vi "fix_shared_library_wildcards.vi"(8 "error in (no error)":errorcluster, 11 "UnpackedPackage in":refnum<class "PackageFile.lvclass">) -> (0 "error out":errorcluster, 2 "map of replacements made":map{path, path}(c390), 3 "UnpackedPackage out":refnum<class "PackageFile.lvclass">)   [LabVIEW 2020, in "vi_package_building_extensions.lvlib" / "PackageFile.lvclass"]
uses:
  PackageFile.lvclass
  PackageFile.lvclass/PackageFile.ctl
  Extensions/fix_shared_library_wildcards.lvlib
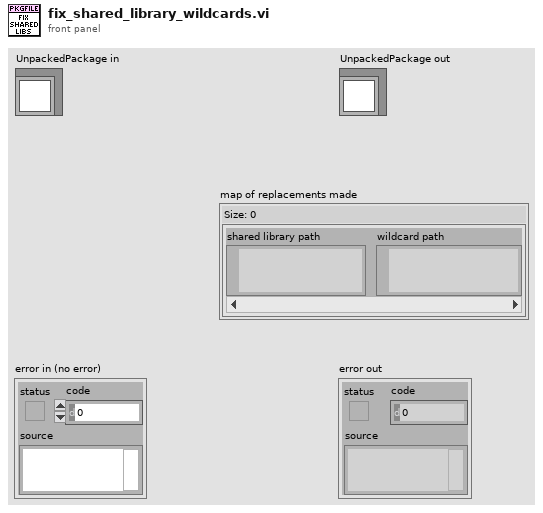
[diagram p1: front panel]
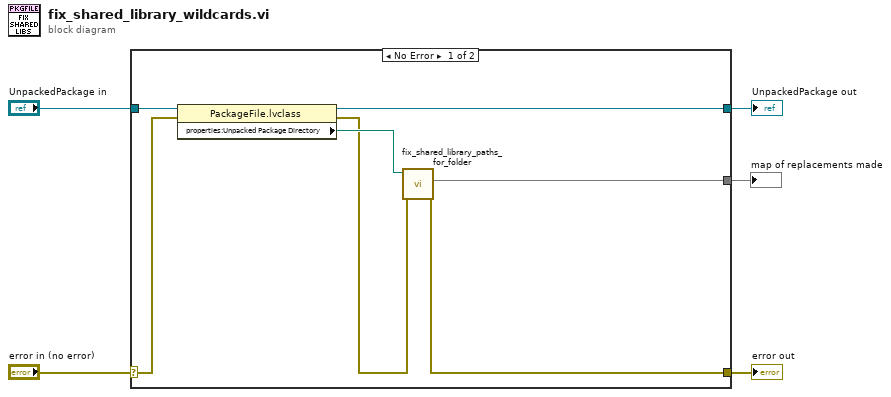
[diagram p0: block diagram]
diagram:
  n1 = case shown="No Error" "error in (no error)" {
    selector: "error in (no error)" -> [w7 w14]
    tunnel: [w11 w14] -> w4
    tunnel: [w9 w13] -> w2
    tunnel: "UnpackedPackage in" -> [w12 w13]
    tunnel: [w10 _] -> w1
    frame No Error {
      n2 = property class="PackageFile.lvclass"(reference=w12, error in=w7) -> (reference out=w9:refnum<class "PackageFile.lvclass">, error out=w6:errorcluster, "properties:Unpacked Package Directory"=w8:path)
      n3 = call "fix_shared_library_paths_for_folder.vi"("error in"=w6, "Folder of VIs"=w8) -> ("error out"=w11:errorcluster, "map of replacements"=w10:map{path, path})  [unwired: 8 in]
    }
    frame Error {
    }
  }
  "error out" <- w4
  "UnpackedPackage out" <- w2
  "map of replacements made" <- w1
